vi "FAMM-service.vi"(8 "error in (no error)":errorcluster, 11 "FAMM_in":refnum<class "FAMM.lvclass">) -> (0 "error out":errorcluster, 3 "FAMM_out":refnum<class "FAMM.lvclass">)   [LabVIEW 2020, in "Sgraph_lib_V1.lvlib" / "FAMM.lvclass"]
doc: "The FAMM server is instantiated by Gserver\nThe FAMM server will process all queue driven commands to read and write from memory, and via the FAMM server access memory or database content.\n\nWhether RAM or Database content is accessed is decided by the FAMM service. Database content is not intended to be accessed directly without using the FAMM service."
uses:
  FAMM.lvclass
  Gserver/controls/Typedef_Gviewer-Query.ctl
  Gserver/controls/Typedef_QueryType.ctl
  HISW/controls/typedef-DAQ-datagram.ctl
  HISW/controls/typedef-Qtype.ctl
  FAMM.lvclass/FAMM.ctl
  controls/FAMMrequest.ctl
  Gview/controls/Typedef_Live.ctl
  Builds/Sgraph_lib_V1.lvlib
  Gview/Gviewer.lvclass
  Gserver/Gserver.lvclass
panel:
  in  "Database_path":path=path "D:/Sgraph_database"
  out "Layers":i32
  out "sec resolution":dbl format="%#_3p"
  out "37x37":picture
  in  "DAQ-Queue":refnum<queue>
  in  "Gserver-Queue":refnum<queue>
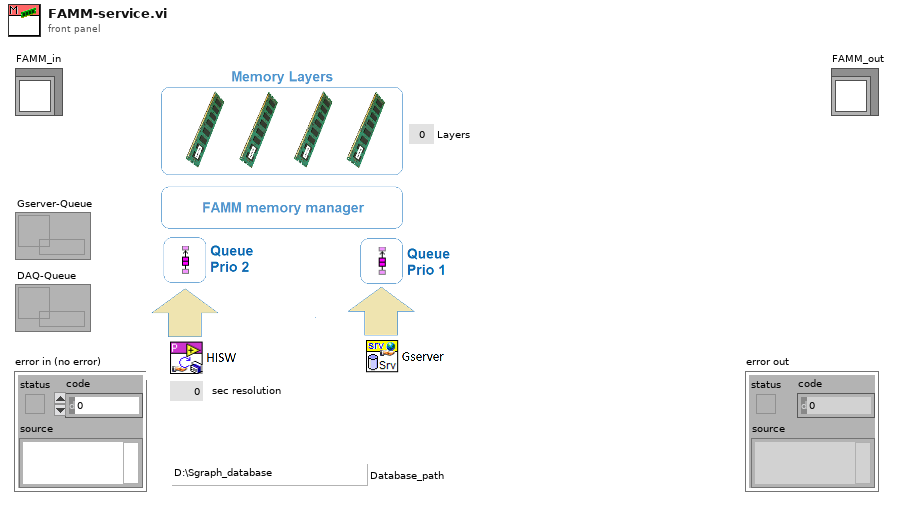
[diagram p1: front panel]
types:
  T1 = typedef "Sgraph_lib_V1.lvlib/FAMM.lvclass/FAMMrequest.ctl" = cluster{"Tags":string[], "Time-Start":timestamp, "Time-End":timestamp, "Live":T2, "TimeSpan":dbl, "DisplayResolution":i32}
  T2 = typedef "Sgraph_lib_V1.lvlib/Gviewer.lvclass/Typedef_Live.ctl" = enum16{"Live View", "Freeze"}
  T3 = typedef "typedef_FAMM_Query.ctl" = cluster{"Time Stamp":timestamp, "FAMM-function":T4, "Source":string, "Data":variant}
  T4 = typedef "typedef-functions.ctl" = enum16{"PAQ-request", "PAQ-taglist-request", "WAQ-request", "EAQ-request", "TAG-based-request", "PAQ-MemoryMap", "Exit-FAMM"}
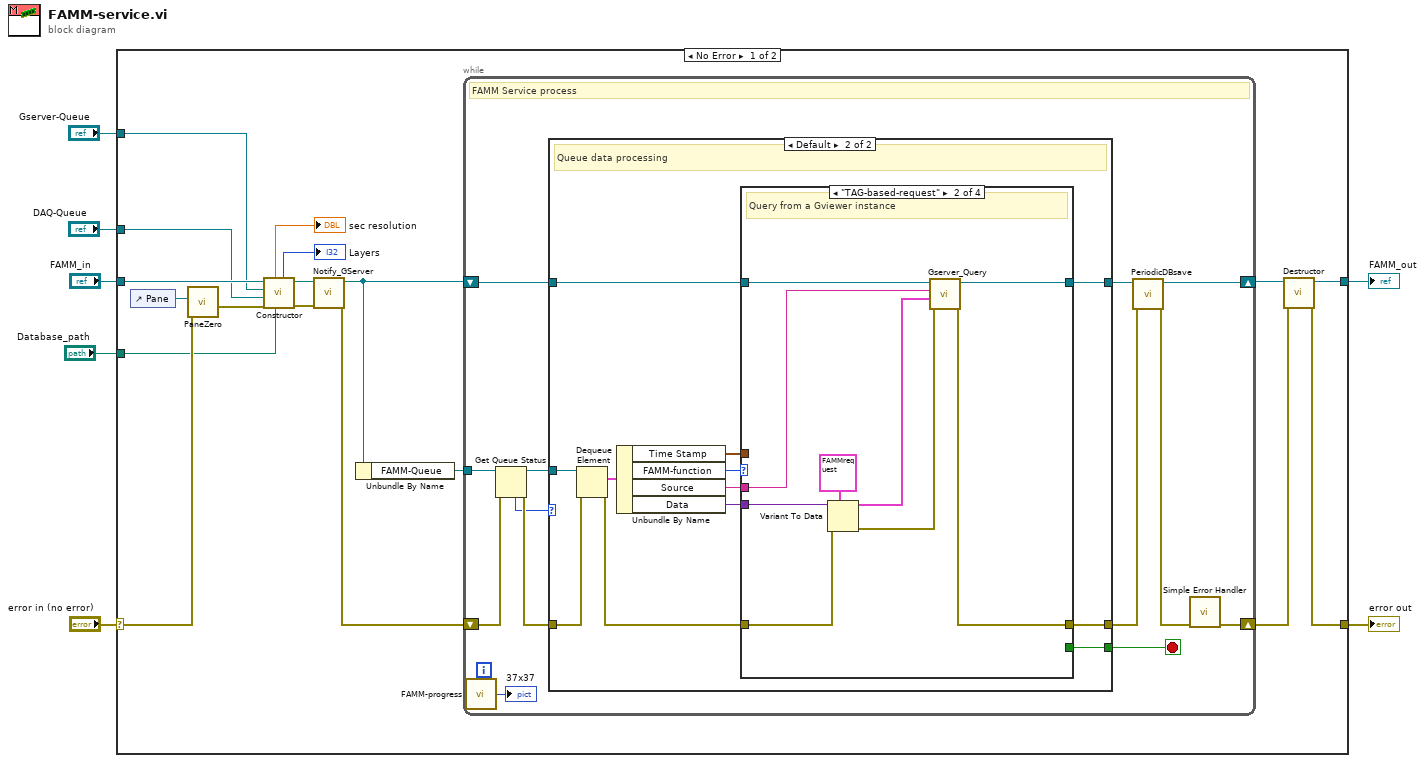
[diagram p0: block diagram]
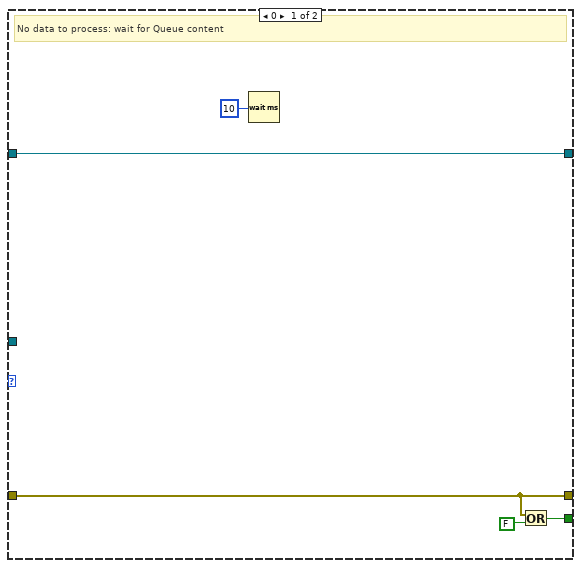
[diagram p2: hidden frame]
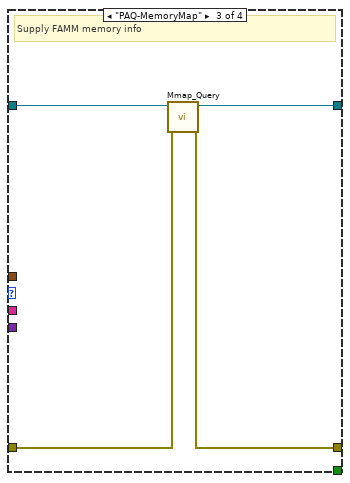
[diagram p4: hidden frame]
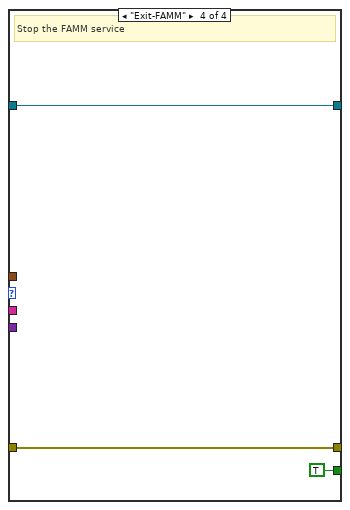
[diagram p5: hidden frame]
diagram:
  n1 = case shown="No Error" "error in (no error)" {
    selector: "error in (no error)" -> [w16 w75]
    tunnel: [w22 w75] -> w6
    tunnel: [w24 w74] -> w5
    tunnel: "FAMM_in" -> [w18 w74]
    tunnel: "Gserver-Queue" -> [w14 _]
    tunnel: "DAQ-Queue" -> [w12 _]
    tunnel: "Database_path" -> [w8 _]
    frame No Error {
      n2 = control-ref of="Pane"() -> (w15:refnum<vi>)
      n3 = call "PaneZero.vi"("error in (no error)"=w16, "Pane"=w15) -> ("error out"=w17:errorcluster)  [unwired: 9 in]
      n4 = call "Constructor.vi"("Database_path"=w8, "error in (no error)"=w17, "DAQ-Queue"=w12, "Gserver-Queue"=w14, "FAMM in"=w18) -> ("error out"=w20:errorcluster, "FAMM out"=w21:refnum<class "FAMM.lvclass">, "Layers"=→"Layers":i32, "Resolution"=→"sec resolution":dbl)  [unwired: 3 in]
      n5 = call "Notify_GServer.vi"("error in (no error)"=w20, "FAMM in"=w21) -> ("error out"=w19:errorcluster, "FAMM out"=w11:refnum<class "FAMM.lvclass">)  [unwired: 8 in]
      n6 = Unbundle By Name(w11) -> ("FAMM-Queue"=w13:refnum<queue>)
      n7 = while {
        shift-right: [w30] -> w25
        shift-left: w11 -> [w31]
        shift-right: [w26] -> w23
        shift-left: w19 -> [w38]
        tunnel: w13 -> [w36]
        stop <- w33 stop-if-true
        # "FAMM Service process"
        n8 = call "FAMM-progress.vi"() -> ("37x37"=→"37x37":picture)  [unwired: 7 in]
        n9 = Get Queue Status(queue=w36, error in (no error)=w38) -> (queue out=w35:refnum<queue>, error out=w37:errorcluster, # elements in queue=w34:i32)  [unwired: 1 in, 5 out]
        n10 = case shown="Default" w34 {
          tunnel: [w39 w55] -> w28
          tunnel: w37 -> [w39 w47]
          tunnel: w31 -> [w41 w54]
          tunnel: [w41 w53] -> w29
          tunnel: w35 -> [_ w52]
          tunnel: [w42 w49] -> w33
          frame 0 {
            # "No data to process: wait for Queue content"
            n11 = Wait (ms)(milliseconds to wait=u32 10) -> ()  [unwired: 1 out]
            n12 = Or(x=w39, y=FALSE) -> (x .or. y?=w42:bool)
          }
          frame Default {
            # "Queue data processing"
            n13 = Dequeue Element(queue=w52, error in (no error)=w47) -> (element=w51:T3, error out=w48:errorcluster)  [unwired: 1 in, 2 out]
            n14 = Unbundle By Name(w51) -> ("Time Stamp"=w44:timestamp, "FAMM-function"=w50:T4, "Source"=w46:string, "Data"=w45:variant)
            n15 = case shown="\"TAG-based-request\"" w50 {
              tunnel: w54 -> [w57 w65 w69 w71]
              tunnel: [w57 w66 w70 w71] -> w53
              tunnel: w48 -> [w56 w61 w68 w73]
              tunnel: [w56 w62 w67 w73] -> w55
              tunnel: [_ _ _ TRUE] -> w49
              tunnel: w46 -> [_ w58 _ _]
              tunnel: w45 -> [_ w64 _ _]
              tunnel: w44 -> [_ _ _ _]
              frame Default {
                # "Not defined"
              }
              frame "TAG-based-request" {
                # "Query from a Gviewer instance"
                n16 = Variant To Data(error in=w61, type=T1 {"Tags"=["ch0001", "ch0002", "ch0003", "ch0004", "ch0005"], "Time-Start"=timestamp(3693712856.876272 s since 1904-01-01), "Time-End"=timestamp(3693716456.876272 s since 1904-01-01), "Live"=enum."Live View", "TimeSpan"=0.0, "DisplayResolution"=0} ("FAMM-request"), Variant=w64) -> (data=w59:T1, error out=w63:errorcluster)
                n17 = call "Gserver_Query.vi"("error in (no error)"=w63, "Query"=w59, "Requester"=w58, "FAMM in"=w65) -> ("error out"=w62:errorcluster, "FAMM out"=w66:refnum<class "FAMM.lvclass">)  [unwired: 6 in]
              }
              frame "PAQ-MemoryMap" {
                # "Supply FAMM memory info"
                n18 = call "Mmap_Query.vi"("error in (no error)"=w68, "FAMM in"=w69) -> ("error out"=w67:errorcluster, "FAMM out"=w70:refnum<class "FAMM.lvclass">)  [unwired: 8 in]
              }
              frame "Exit-FAMM" {
                # "Stop the FAMM service"
              }
            }
          }
        }
        n19 = call "PeriodicDBsave.vi"("error in (no error)"=w28, "FAMM in"=w29) -> ("error out"=w27:errorcluster, "FAMM out"=w30:refnum<class "FAMM.lvclass">)  [unwired: 8 in]
        n20 = call <vilib>:"Simple Error Handler.vi"("error in (no error)"=w27) -> ("error out"=w26:errorcluster)  [unwired: 4 in, 4 out]
      }
      n21 = call "Destructor.vi"("error in (no error)"=w23, "FAMM in"=w25) -> ("error out"=w22:errorcluster, "FAMM out"=w24:refnum<class "FAMM.lvclass">)  [unwired: 8 in]
    }
    frame Error {
    }
  }
  "error out" <- w6
  "FAMM_out" <- w5
